vi "Lire config KELLER.vi"(2 "error in (no error)":errorcluster caption="entrée d'erreur (pas d'erreur)", 3 "refnum":T1) -> (0 "error out":errorcluster, 1 "refnum out":T1)   [LabVIEW 2022 SP3]
uses:
  <vilib>/Utility/config.llb/Config Data RefNum.ctl
  <vilib>/Utility/config.llb/Read Key (String).vi
  <vilib>/Utility/config.llb/Read Key (Boolean).vi
  Variables globales/Variable glob Keller.vi
  <vilib>/Utility/config.llb/NI_LVConfig.lvlib
panel:
  out "Sélections KELLER":bool[](array[boolean])
  out "Port COM KELLER":refnum<visa-resource-name>="COM7"
  out "Adresses KELLER":u8[](array[numeric])=[1, 1] max=6
  out "Noms capteurs KELLER":string[](array[string])
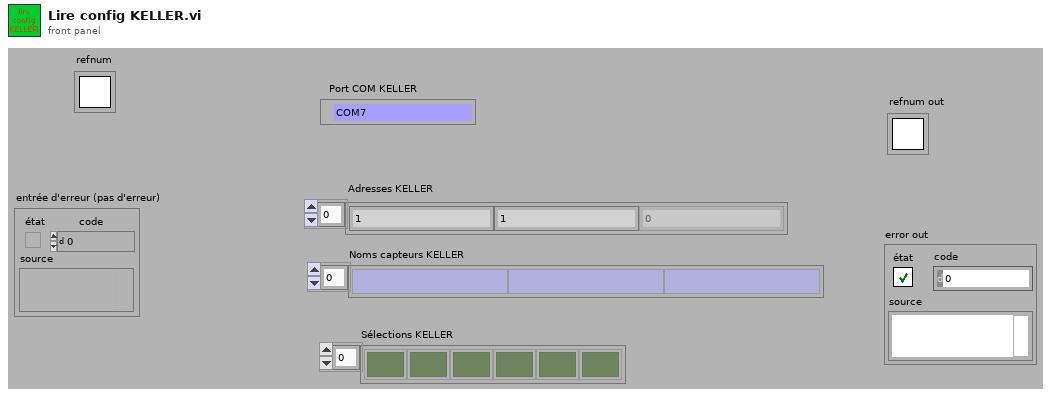
[diagram p1: front panel]
types:
  T1 = typedef "NI_LVConfig.lvlib/Config Data RefNum.ctl" = refnum<k1>
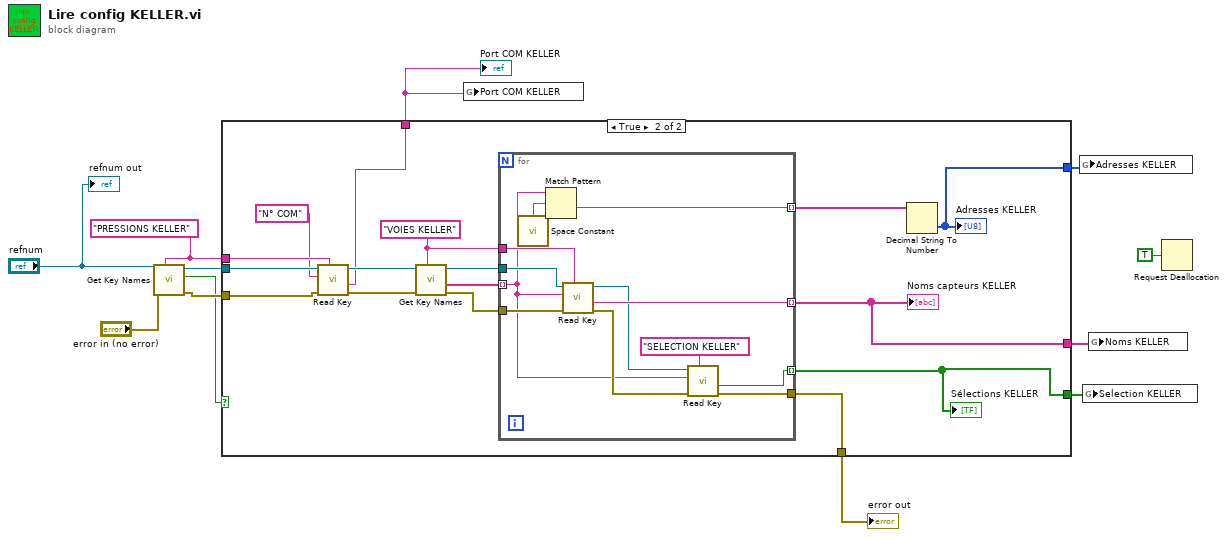
[diagram p0: block diagram]
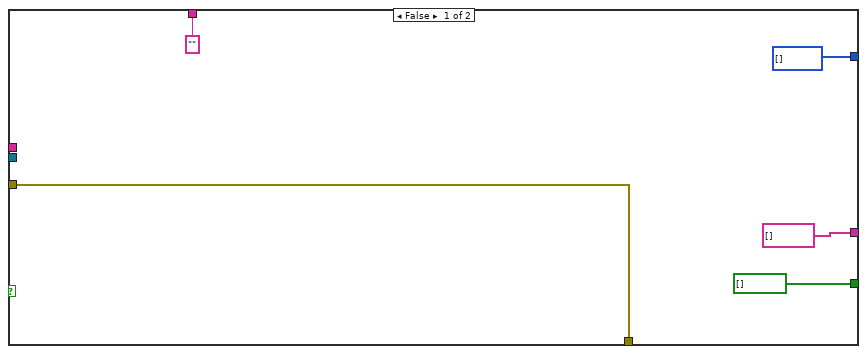
[diagram p2: hidden frame]
diagram:
  w10 = "PRESSIONS KELLER" ("section")
  n1 = call <vilib>:"Get Key Names.vi"("section"=w10, "error in (no error)"="error in (no error)", "refnum"="refnum") -> ("error out"=w11:errorcluster, "section exists?"=w7:bool, "refnum out"=w12:T1)  [unwired: 5 in, 1 out]
  n2 = case shown="True" w7 {
    tunnel: w12 -> [_ w33]
    tunnel: w11 -> [w13 w32]
    tunnel: w10 -> [_ w31]
    tunnel: [w13 w21] -> w9
    tunnel: ["" ("value") w19] -> w6
    tunnel: [i32[] [] w22] -> w5
    tunnel: [string[] [] w23] -> w4
    tunnel: [bool[] [] w18] -> w3
    frame False {
    }
    frame True {
      w20 = "VOIES KELLER" ("section")
      n3 = call-poly <vilib>:"Read Key.vi"("section"=w31, "error in (no error)"=w32, "key"="N° COM", "refnum"=w33) -> ("error out"=w30:errorcluster, "value"=w19:string, "refnum out"=w29:T1)  [unwired: 4 in, 1 out]
      n4 = call <vilib>:"Get Key Names.vi"("section"=w20, "error in (no error)"=w30, "refnum"=w29) -> ("error out"=w25:errorcluster, "key names"=w27:string[], "refnum out"=w26:T1)  [unwired: 5 in, 1 out]
      n5 = for {
        tunnel: w27 -> [w35] mode=indexing
        tunnel: w26 -> [w45]
        tunnel: w25 -> [w44]
        tunnel: [w43] -> w23 mode=indexing
        tunnel: [w41] -> w24 mode=indexing
        tunnel: [w37] -> w21
        tunnel: w20 -> [w40]
        tunnel: [w34] -> w18 mode=indexing
        n6 = call <vilib>:"Space Constant.vi"() -> ("String"=w42:string)
        n7 = Match Pattern(string=w35, regular expression=w42) -> (after substring=w41:string)  [unwired: 1 in, 3 out]
        n8 = call-poly <vilib>:"Read Key.vi"("section"=w40, "error in (no error)"=w44, "key"=w35, "refnum"=w45) -> ("error out"=w38:errorcluster, "value"=w43:string, "refnum out"=w39:T1)  [unwired: 4 in, 1 out]
        n9 = call-poly <vilib>:"Read Key.vi"("section"="SELECTION KELLER", "error in (no error)"=w38, "key"=w35, "refnum"=w39) -> ("error out"=w37:errorcluster, "value"=w34:bool)  [unwired: 4 in, 2 out]
      }
      "Noms capteurs KELLER" <- w23
      "Sélections KELLER" <- w18
      n10 = Decimal String To Number(string=w24) -> (number=w22:i32[])  [unwired: 2 in, 1 out]
      "Adresses KELLER" <- w22
    }
  }
  "error out" <- w9
  "Port COM KELLER" <- w6
  n11 = global write "Variable glob Keller.vi" "Port COM KELLER"(w6) -> ()
  n12 = global write "Variable glob Keller.vi" "Adresses KELLER"(w5) -> ()
  n13 = global write "Variable glob Keller.vi" "Selection KELLER"(w3) -> ()
  n14 = global write "Variable glob Keller.vi" "Noms KELLER"(w4) -> ()
  n15 = Request Deallocation(TRUE ("flag")) -> ()
  "refnum out" <- "refnum"
